vi "D_Mode_Select.vi"(8 "error in (no error)":errorcluster, 10 "mode":u8, 11 "bID":u8) -> (0 "error out":errorcluster, 3 "bID":u8, 4 "TorF":i32)   [LabVIEW 2013]
uses:
  LabVIEW2018/hpkSLMdaLV.dll
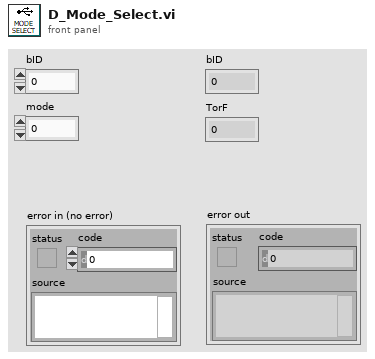
[diagram p1: front panel]
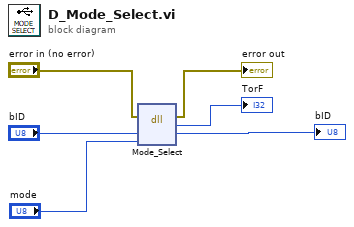
[diagram p0: block diagram]
diagram:
  n1 = dll-call lib="C:/Users/hs5921/Desktop/LabVIEW2018/hpkSLMdaLV.dll" fn="Mode_Select"(error in="error in (no error)", "bID"="bID", "mode"="mode") -> (error out=→"error out":errorcluster, "返り値タイプ"=→"TorF":i32, "bID"=→"bID":u8)  [unwired: 3 in, 1 out]
